vi "SMTP Email Format Text Message.vi"(5 "translit":string, 6 "character set":string caption="jeu de caractères", 7 "last chunk (T)":bool=TRUE caption="dernière partie (V)", 8 "prev data (\"\")":string caption="donnée préc (\"\")", 9 "text":string caption="texte") -> (0 "real charset":string caption="jeu de caractères réel", 2 "next data":string caption="donnée suivante", 3 "formated text":string caption="texte formaté")   [LabVIEW 2022 SP3, in "Copie de NI_SMTPEmail.lvlib"]
doc: "Ce VI prend un message texte (ou une grande partie de celui-ci) et le rend conforme à MIME si bien qu'il peut être envoyé sur Internet grâce au protocole SMTP. Ce VI utilise des encodages annoncés affichables pour l'ensemble de caractère étendu. Le paramètre Dernière partie est utilisé quand une large quantitié de données doit être envoyées (par exemple quand on lit les données d'un fichier). De ce cas, on peut convertir les données par blocs. Cependant, pour que le VI puisse tout assembler correctement, il doit conserver l'état des blocs. Donc, quand le dernier bloc a été envoyé, le paramètre Dernière partie doit être défini à VRAI"
uses:
  Copie de NI_SMTPEmail.lvlib
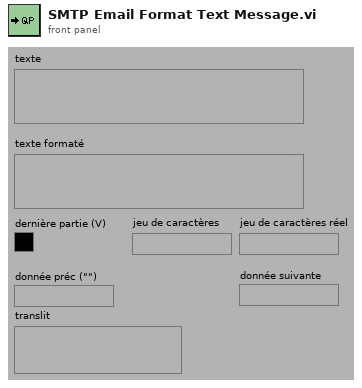
[diagram p1: front panel]
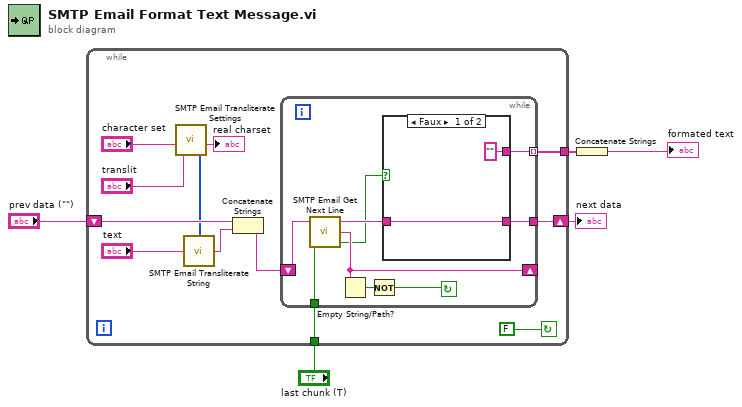
[diagram p0: block diagram]
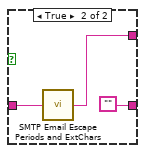
[diagram p2: hidden frame]
diagram:
  n1 = while {
    tunnel: "last chunk (T)" -> [w8]
    tunnel: [w9] -> w5
    shift-left: "prev data (\"\")" -> [w15]
    shift-right: [w16] -> w3
    stop <- FALSE continue-if-true
    n2 = call "SMTP Email Transliterate Settings.vi"("transliteration"="translit", "character set"="character set") -> ("map"=w14:u8[], "charset out"=→"real charset":string)  [unwired: 4 in]
    n3 = call "SMTP Email Transliterate String.vi"("text in"="text", "map"=w14) -> ("text out"=w13:string)
    n4 = Concatenate Strings(w15, w13) -> (w17:string)
    n5 = while {
      tunnel: w8 -> [w18]
      tunnel: [w25] -> w9 mode=indexing
      shift-left: w17 -> [w20]
      shift-right: [w23] -> _
      tunnel: [w26] -> w16
      stop <- w21 continue-if-true
      n6 = call "SMTP Email Get Next Line.vi"("last chunk"=w18, "string"=w20) -> ("found eoln"=w19:bool, "after eoln"=w23:string, "before eoln"=w24:string)  [unwired: 1 in]
      n7 = Empty String/Path?(string/path=w23) -> (empty?=w22:bool)
      n8 = Not(x=w22) -> (.not. x?=w21:bool)
      n9 = case shown="Faux" w19 {
        tunnel: ["" ("Formatted Line of Text") w29] -> w25
        tunnel: w24 -> [w28 w30]
        tunnel: [w28 ""] -> w26
        frame False {
        }
        frame True {
          n10 = call "SMTP Email Escape Periods and ExtChars.vi"("string"=w30) -> ("quoted string"=w29:string)
        }
      }
    }
  }
  "next data" <- w3
  n11 = Concatenate Strings(w5) -> (→"formated text":string)
